vi "CalcExpress - Eval Script.vi"(5 "VC Handle":T3=-1, 6 "error in":bool, 7 "params":T2={"autoVar"=TRUE, "enCpx"=TRUE}, 8 "repeat (1)":i32=1, 9 "CE InstanceRef":T1) -> (0 "error out":bool, 1 "value type":T4=enum."DBL Number", 2 "numeric value":dbl, 3 "dup CE InstanceRef":T1, 4 "dup VC Handle":T3=-1)   [LabVIEW 2021]
doc: "The VI evaluates previously parsed CalcExpress expressions and sequential scripts. To process non-sequential scripts involving loops and branches, use CSE VIs.\n\nThis basic (low-level) VI has boolean error connectors instead of traditional error clusters. For more convenience, you can use top-level CalcExpress VIs that use error clusters.\n\nFor more information, see help for this VI.\n\n::: CalcExpress Toolkit :::\nCopyright (c) 2000-2026 Konstantin Shifershteyn. All rights reserved."
uses:
  cetypes.llb/VarMan Variable Context Handle.ctl
  cetypes.llb/CalcExpress Data Type.ctl
  cetypes.llb/CalcExpress Execution Options.ctl
  cetypes.llb/CalcExpress Instance RefNum.ctl
  cersrc/celveng32.dll
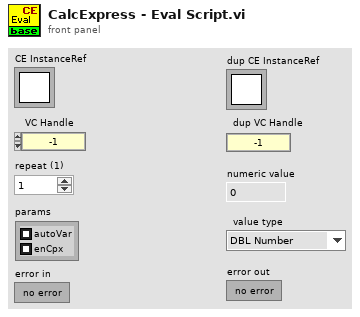
[diagram p1: front panel]
types:
  T1 = typedef "CalcExpress Instance RefNum.ctl" = refnum<k1>
  T2 = typedef "CalcExpress Execution Options.ctl" = cluster{"autoVar":bool, "enCpx":bool}
  T3 = typedef "VarMan Variable Context Handle.ctl" = i32
  T4 = typedef "CalcExpress Data Type.ctl" = enum32{"String", "DBL Number", "identifier", "1D Array of DBL", "2D Array of DBL", "CDB Number", "1D Array of CDB", "2D Array of CDB", "1D Array of String", "2D Array of String", "Unknown data type"}
  T5 = enum32{"String", "DBL Number", "identifier", "1D Array of DBL", "2D Array of DBL", "CDB Number", "1D Array of CDB", "2D Array of CDB", "1D Array of String", "2D Array of String", "Unknown data type"}
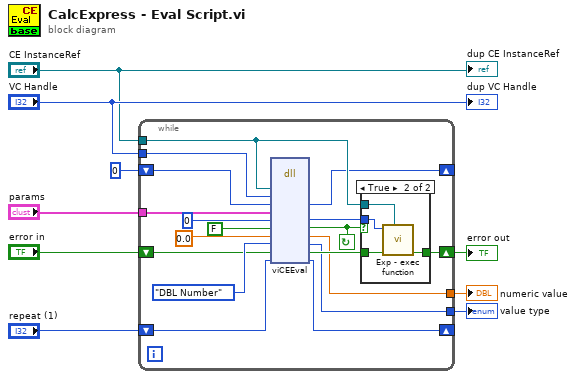
[diagram p0: block diagram]
diagram:
  n1 = while {
    shift-left: "repeat (1)" -> [w17]
    shift-right: [w16] -> _
    tunnel: [w14] -> w3
    tunnel: [w13] -> w4
    tunnel: "VC Handle" -> [w25]
    tunnel: "CE InstanceRef" -> [w26]
    tunnel: "params" -> [w23]
    shift-left: 0 -> [w24]
    shift-right: [w10] -> _
    shift-left: "error in" -> [w18]
    shift-right: [w27] -> w5
    stop <- w12 continue-if-true
    n2 = dll-call lib="C:/LV Projects/CalcExpress 40 LV2021/vi.lib/addons/CalcExpress/cersrc/celveng*.dll" fn="viCEEval"("iRef"=w26, "vch"=w25, "idx"=w24, "cPars"=w23, "opdNum"=0, "NE"=FALSE, "num"=0.0 ("numeric value"), "type"=T5."DBL Number" ("data type"), "erf"=w18, "rept"=w17) -> ("idx"=w10:i32, "opdNum"=w11:i32, "NE"=w12:bool, "num"=w13:dbl, "type"=w14:T5, "erf"=w15:bool, "rept"=w16:i32)  [unwired: 7 in, 2 out]
    n3 = case shown="True" w12 {
      tunnel: [w28 w32] -> w27
      tunnel: w15 -> [w28 w31]
      tunnel: w11 -> [_ w30]
      tunnel: w26 -> [_ w29]
      frame False {
      }
      frame True {
        n4 = call "Exp - exec function.vi"("CE InstanceRef"=w29, "error in"=w31, "ParNum"=w30) -> ("error out"=w32:bool)  [unwired: 6 in]
      }
    }
  }
  "error out" <- w5
  "numeric value" <- w4
  "value type" <- w3
  "dup VC Handle" <- "VC Handle"
  "dup CE InstanceRef" <- "CE InstanceRef"
